vi "MODBUSDATOSPID.vi"() -> ()   [LabVIEW 2023]
uses:
  <vilib>/Modbus/master/Create Master Instance (TCP).vi
  <vilib>/addons/control/pid/pid.llb/PID (DBL).vi
  <vilib>/Modbus/master/Modbus Master.lvclass
  <vilib>/addons/control/pid/NI_PID_pid.lvlib
panel:
  in  "setpoint":dbl
  in  "output range":cluster{"output high":dbl, "output low":dbl}={"output high"=100.0, "output low"=-100.0} {"output low" format="%.2f"; "output high" format="%.2f"}
  in  "PID gains":T1={"proportional gain (Kc)"=922.0, "integral time (Ti, min)"=276.0, "derivative time (Td, min)"=768.0} {"derivative time (Td, min)" format="%.3f"; "integral time (Ti, min)" format="%.3f"; "proportional gain (Kc)" format="%.3f"}
  out "muestreo":u32
  in  "address":string="192.168.1.6"
  out "Waveform Chart":dbl(graph)
  out "FLUJO":dbl(knob) scale=0.0..10.0
  out "NIVEL":dbl(slide) scale=0.0..10.0
  in  "Vaciado":u16(slide) scale=0.0..100.0
  in  "Llenado":u16(slide) scale=0.0..100.0
  in  "stop":bool
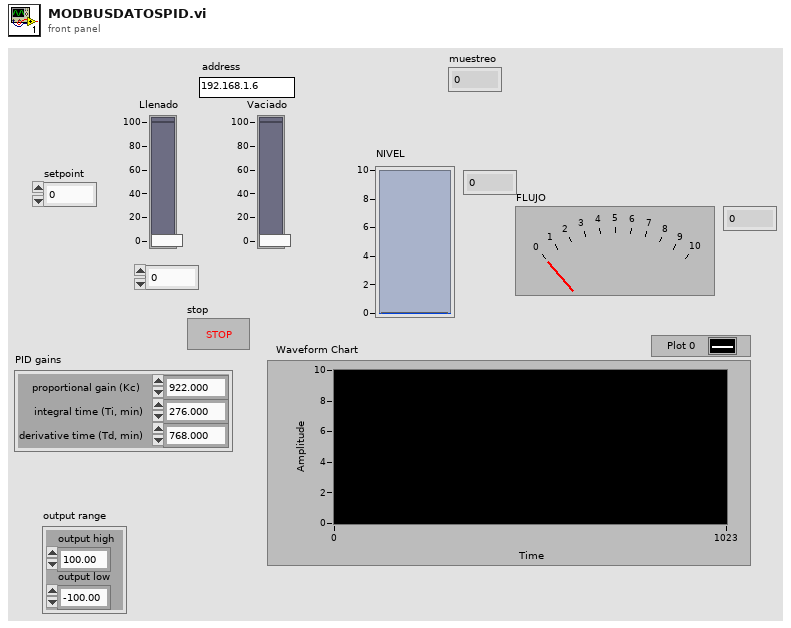
[diagram p1: front panel]
types:
  T1 = cluster{"proportional gain (Kc)":dbl, "integral time (Ti, min)":dbl, "derivative time (Td, min)":dbl}
  T2 = enum16{"open", "replace", "create", "open or create", "replace or create", "replace or create with confirmation"}
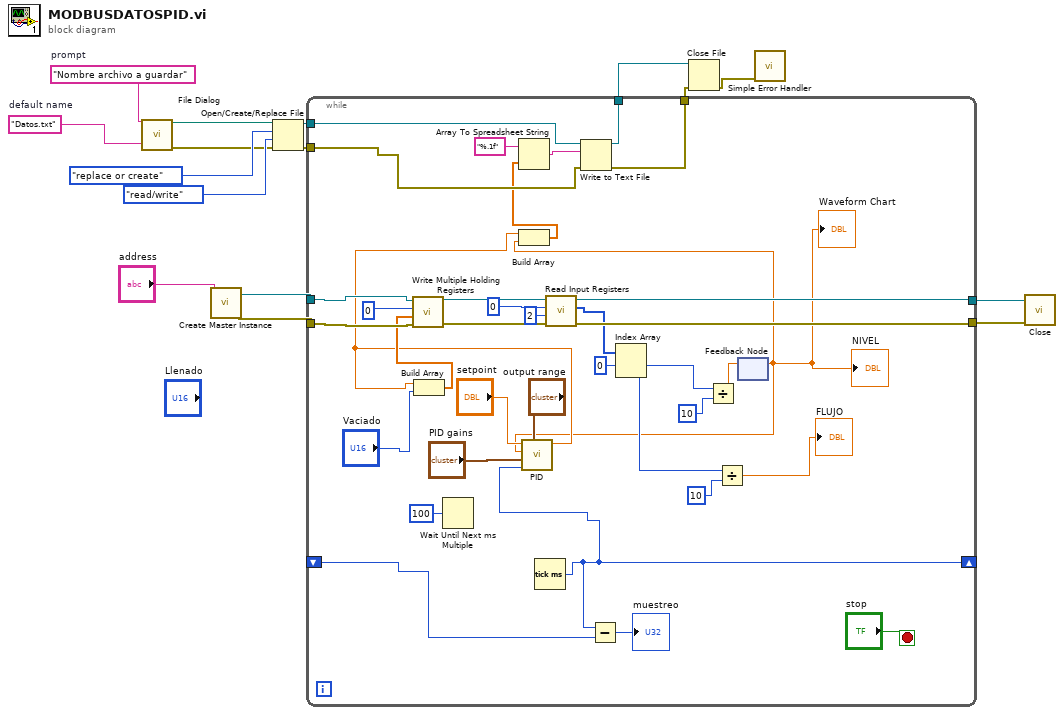
[diagram p0: block diagram]
diagram:
  w12 = "Datos.txt"  # default name
  w7 = "Nombre archivo a guardar"  # prompt
  n1 = call "File Dialog"("prompt"=w7, "pattern (all files)"=w12) -> ("selected path"=w9:path, "error out"=w8:errorcluster)  [unwired: 10 in, 2 out]
  n2 = call-poly <vilib>:"Create Master Instance.vi"("address"="address") -> ("error out"=w15:errorcluster, "TCP master instance"=w16:refnum<class "Modbus Master.lvclass">)  [unwired: 9 in]
  n3 = Open/Create/Replace File(file path (use dialog)=w9, error in=w8, operation (0:open)=T2."replace or create", access (0:read/write)=enum16{"read/write", "read-only", "write-only"}."read/write") -> (refnum out=w6:refnum<file>, error out=w5:errorcluster)  [unwired: 2 in, 1 out]
  n4 = while {
    tunnel: w16 -> [w51]
    tunnel: w15 -> [w49]
    tunnel: [w42] -> w14
    tunnel: [w41] -> w13
    tunnel: w6 -> [w31]
    tunnel: w5 -> [w30]
    tunnel: [w29] -> w3
    tunnel: [w28] -> w2
    shift-right: [w23] -> _
    shift-left: _ -> [w26]
    stop <- "stop" stop-if-true
    n5 = Wait Until Next ms Multiple(millisecond multiple=u32 100) -> ()  [unwired: 1 out]
    n6 = Tick Count (ms)() -> (millisecond timer value=w23:u32)
    n7 = Subtract(x=w23, y=w26) -> (x-y=→"muestreo":u32)
    n8 = feedback #1() -> (w17:dbl)  [unwired: 1 in]
    "NIVEL" <- w17
    "Waveform Chart" <- w17
    n9 = call-poly <vilib>:"PID.vi"("output range"="output range", "dt (s)"=w23, "PID gains"="PID gains", "process variable"=w17, "setpoint"="setpoint") -> ("output"=w20:dbl)  [unwired: 5 in, 1 out]
    n10 = Build Array(w20, "Vaciado") -> (w47:dbl[])
    n11 = call-dynamic "Write Multiple Holding Registers.vi"("error in (no error)"=w49, "holding register values"=w47, "starting address"=u16 0, "Modbus master in"=w51) -> ("error out"=w45:errorcluster, "Modbus master out"=w46:refnum<class "Modbus Master.lvclass">)  [unwired: 6 in]
    n12 = Build Array(w20, w17) -> (w27:dbl[])
    n13 = Array To Spreadsheet String(array=w27, 3:"%.1f") -> (spreadsheet string=w33:string)  [unwired: 1 in]
    n14 = call-dynamic "Read Input Registers.vi"("error in (no error)"=w45, "number of input registers"=u16 2, "starting address"=u16 0, "Modbus master in"=w46) -> ("error out"=w41:errorcluster, "register values"=w40:u16[], "Modbus master out"=w42:refnum<class "Modbus Master.lvclass">)  [unwired: 5 in]
    n15 = Write to Text File(file (use dialog)=w31, text=w33, error in=w30) -> (refnum out=w28:refnum<file>, error out=w29:errorcluster)  [unwired: 1 in, 1 out]
    n16 = Index Array(array=w40, index #1=0 ("index")) -> (element #1=w38:u16, element #2=w35:u16)  [unwired: 1 in]
    n17 = Divide(x=w38, y=u16 10) -> (x/y=w18:dbl)
    n18 = Divide(x=w35, y=u16 10) -> (x/y=→"FLUJO":dbl)
    n19 = feedback-in #1(w18) -> ()
  }
  n20 = Close File(refnum=w2, error in=w3) -> (error out=w4:errorcluster)  [unwired: 1 out]
  n21 = call <vilib>:"Simple Error Handler.vi"("error in (no error)"=w4) -> ()  [unwired: 4 in, 5 out]
  n22 = call-dynamic "Close.vi"("error in (no error)"=w13, "Modbus master in"=w14) -> ()  [unwired: 9 in, 1 out]
